vi "Plot Waypoint Tangent.vi"() -> ()   [LabVIEW 2020]
panel:
  out "T_i":cluster{dbl, dbl}
  in  "point c":cluster{"x":dbl, "y":dbl}
  in  "point b":cluster{"x":dbl, "y":dbl}
  in  "point a":cluster{"x":dbl, "y":dbl}
  out "XY Graph":cluster{cluster{"x":dbl, "y":dbl}[]}[](graph)
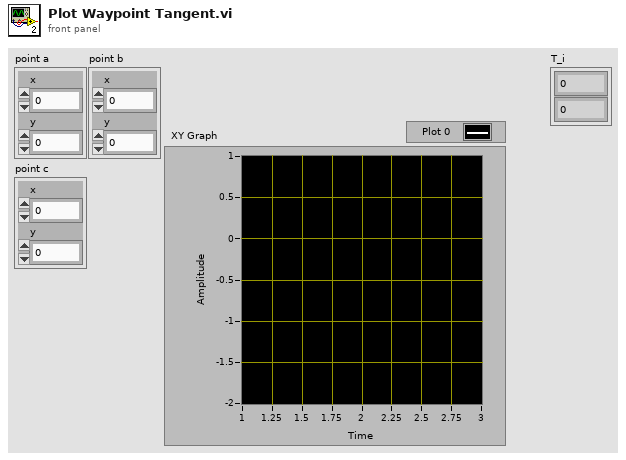
[diagram p1: front panel]
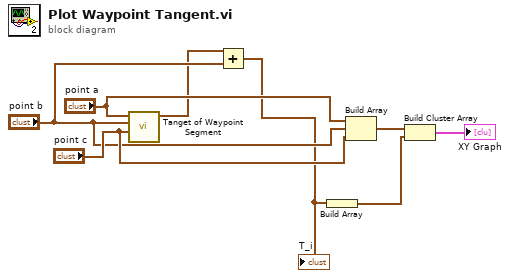
[diagram p0: block diagram]
diagram:
  n1 = call "Tanget of Waypoint Segment.vi"("point c"="point c", "point b"="point b", "point a"="point a") -> ("T_i"=w5:cluster{sgl, sgl})  [unwired: 8 in]
  n2 = Add(x=w5, y="point b") -> (x+y=w3:cluster{dbl, dbl})
  "T_i" <- w3
  n3 = Build Array(w3) -> (w2:cluster{dbl, dbl}[])
  n4 = Build Array("point a", "point b", "point c") -> (w4:cluster{"x":dbl, "y":dbl}[])
  n5 = Build Cluster Array(w4, w2) -> (→"XY Graph":cluster{cluster{"x":dbl, "y":dbl}[]}[])
